vi "addNode.vi"(0 "reference":refnum<class "Graph.lvclass">, 1 "node":refnum<class "AbstractNode.lvclass">, 2 "point":T1 {"y" format="%.2f"; "x" format="%.2f"}, 5 "error in (no error)":errorcluster) -> (14 "reference out":refnum<class "Graph.lvclass">, 19 "error out":errorcluster)   [LabVIEW 2020, in "Graph.lvclass"]
uses:
  <resource>/Framework/Providers/Open_GDS/UML/Graph_class/Graph.lvclass
  <resource>/Framework/Providers/Open_GDS/UML/AbstractNode_class/AbstractNode.lvclass
  <resource>/Framework/Providers/Open_GDS/UML/General/Point/Point Point2D.ctl
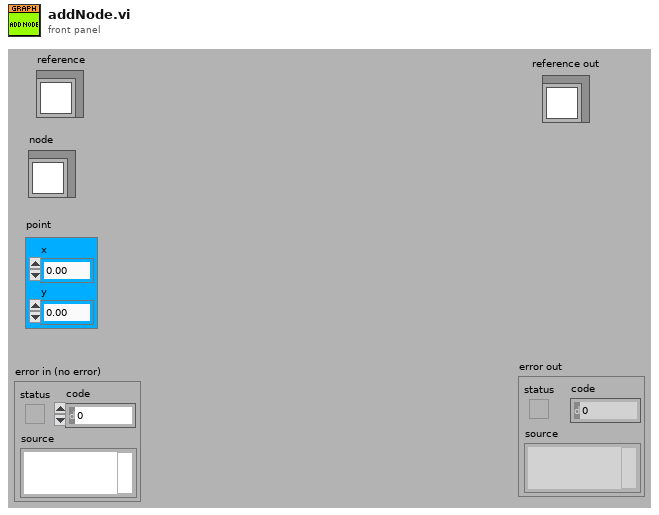
[diagram p1: front panel]
types:
  T1 = typedef "Point Point2D.ctl" = cluster{"x":dbl, "y":dbl}
  T2 = typedef "Rectangle Rectangle2D.ctl" = cluster{"x":dbl, "y":dbl, "width":dbl, "height":dbl}
  T3 = typedef "Graph.lvclass/ObjectAttributes.ctl" = cluster{"nodes":refnum<class "AbstractNode.lvclass">[], "edges":refnum<class "AbstractEdge.lvclass">[], "nodesToBeRemoved":refnum<class "AbstractNode.lvclass">[], "edgesToBeRemoved":refnum<class "AbstractEdge.lvclass">[], "needsLayout":bool, "LayoutNodes":refnum<class "AbstractNode.lvclass">[]}
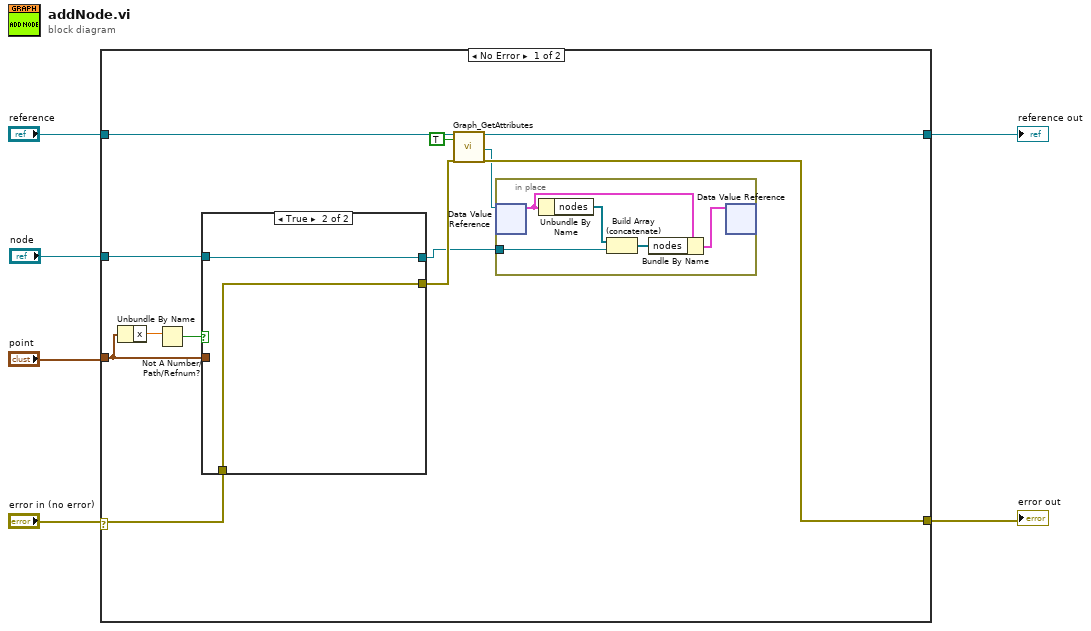
[diagram p0: block diagram]
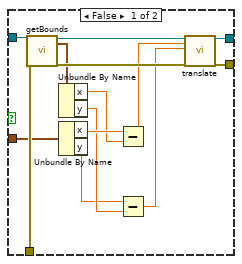
[diagram p2: hidden frame]
diagram:
  n1 = case shown="No Error" "error in (no error)" {
    selector: "error in (no error)" -> [w15 w40]
    tunnel: "reference" -> [w18 w41]
    tunnel: [w17 w40] -> w5
    tunnel: [w16 w41] -> w4
    tunnel: "node" -> [w14 _]
    tunnel: "point" -> [w12 _]
    frame No Error {
      n2 = Unbundle By Name(w12) -> ("x"=w11:dbl)
      n3 = Not A Number/Path/Refnum?(number/path/refnum=w11) -> (NaN/Path/Refnum?=w10:bool)
      n4 = case shown="True" w10 {
        tunnel: w15 -> [w37 w38]
        tunnel: w14 -> [w36 w39]
        tunnel: w12 -> [w35 _]
        tunnel: [w33 w38] -> w13
        tunnel: [w31 w39] -> w7
        frame False {
          n5 = call-dynamic "getBounds.vi"("reference"=w36, "error in (no error)"=w37) -> ("reference out"=w32:refnum<class "AbstractNode.lvclass">, "bounds"=w30:T2, "error out"=w34:errorcluster)  [unwired: 15 in]
          n6 = Unbundle By Name(w30) -> ("x"=w28:dbl, "y"=w27:dbl)
          n7 = Unbundle By Name(w35) -> ("x"=w29:dbl, "y"=w26:dbl)
          n8 = Subtract(x=w29, y=w28) -> (x-y=w24:dbl)
          n9 = Subtract(x=w26, y=w27) -> (x-y=w25:dbl)
          n10 = call-dynamic "translate.vi"("reference"=w32, "dx"=w24, "dy"=w25, "error in (no error)"=w34) -> ("reference out"=w31:refnum<class "AbstractNode.lvclass">, "error out"=w33:errorcluster)  [unwired: 14 in]
        }
        frame True {
        }
      }
      n11 = call <resource>:"Graph_GetAttributes.vi"("reference in"=w18, "OnlyGetDvrReference(False)"=TRUE, "error in (no error)"=w13) -> ("reference out"=w16:refnum<class "Graph.lvclass">, "DataRef"=w8:refnum<data-value>, "error out"=w17:errorcluster)  [unwired: 13 in, 1 out]
      n12 = in-place {
        in-place-border: w7 -> [w19]
        n13 = in-place-dvr #1(w8) -> (w23:T3)  [unwired: 1 out]
        n14 = Unbundle By Name(w23) -> ("nodes"=w20:refnum<class "AbstractNode.lvclass">[])
        n15 = Build Array (concatenate)(w20, w19) -> (w22:refnum<class "AbstractNode.lvclass">[])
        n16 = Bundle By Name(cluster=w23, "nodes"=w22) -> (w21:T3)
        n17 = in-place-dvr #1(w21) -> ()  [unwired: 2 out]
      }
    }
    frame Error {
    }
  }
  "reference out" <- w4
  "error out" <- w5
